vi "Write String.vi"(8 "error in (no error)":errorcluster, 9 "Timeout (ms)":i32, 10 "Data":string, 11 "CIFTag in":refnum<class "CIF_Iceoryx_Chn_String.lvclass">) -> (0 "error out":errorcluster, 1 "timed out?":bool, 3 "CIFTag out":refnum<class "CIF_Iceoryx_Chn_String.lvclass">)   [LabVIEW 2021, in "CIF_Iceoryx_Chn_String.lvclass"]
uses:
  CIF_Iceoryx_Chn_String.lvclass
  D:/dev/Packages/CIF_Channels_Core/src/CIFChannels/CIFChannels.lvclass
  D:/dev/Packages/CIF_Channels_Core/src/Iceorxy_Channels/CIF_Iceoryx_BB/CIF_Iceoryx_BB.lvclass
  CIFChannels/CIFChannels.lvclass/CIFChannels.ctl
  CIF_Iceoryx_Chn_String.lvclass/CIF_Iceoryx_Chn_String.ctl
  CIF_Iceoryx_BB/CIF_Iceoryx_BB.lvclass/CIF_Iceoryx_BB.ctl
  <vilib>/Utility/error.llb/Clear Errors.vi
  ChannelCommon/Utilities/Add Error.vi
  CIF_Iceoryx_BB/Accessors/Read Writer Reference.vi
  Write String Direct.vi/46c631c6-c319-459f-b22a-b0c63d4769f6.vi
  CIFChannels/Accessors/Read Tag Forced.vi
  <vilib>/CIF Foundation/CIF Iceoryx/SubVIs/Get Path.vi
  <vilib>/CIF Foundation/CIF Iceoryx/SubVIs/Convert Error.vi
  <vilib>/CIF Foundation/CIF Iceoryx/Refnum/BB Writer from Refnum.vi
  <vilib>/CIF Foundation/CIF Iceoryx/SubVIs/Convert Error Core.vi
  ChannelCommon/Utilities/Add Error Core.vi
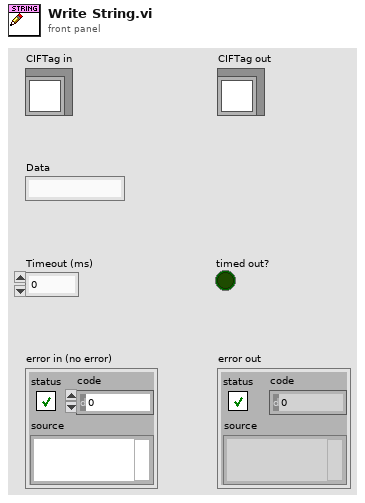
[diagram p1: front panel]
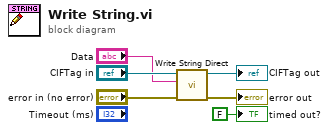
[diagram p0: block diagram]
diagram:
  n1 = call "Write String Direct.vi"("error in (no error)"="error in (no error)", "Data"="Data", "CIFTag in"="CIFTag in") -> ("error out"=→"error out":errorcluster, "CIFTag out"=→"CIFTag out":refnum<class "CIF_Iceoryx_Chn_String.lvclass">)  [unwired: 7 in]
  "timed out?" <- FALSE ("timed out?")
